vi "Mark Tool Error Result.vi"(8 "error in":errorcluster, 11 "response":string) -> (0 "error out":errorcluster, 3 "response out":string)   [LabVIEW 2020, in "MCP Server.lvlib"]
doc: "Marks the result of tools/call as a tool execution error when the tool VI itself reported an error.\n\nThe outputs of the tool are returned as one JSON object in the first text item of content. If one of the outputs is an error cluster (an object with status, code and source) whose status is true, the result gets \"isError\": true. The content is not changed.\n\nEvery other response is passed through."
uses:
  MCP Server.lvlib
  5611462b-074d-46fb-9f1a-e631b5fec0f0.vi
  <vilib>/JDP Science/JSONtext/Next JSON Value.vi
  <vilib>/JDP Science/JSONtext/String Subset.vi
  <vilib>/JDP Science/JSONtext/Parsing/Advance past next JSON Value (inlined COPY).vi
  <vilib>/JDP Science/JSONtext/Parsing/Advance past whitespace.vi
  <vilib>/JDP Science/JSONtext/Parsing/Advance past String.vi
  <vilib>/JDP Science/JSONtext/Parsing/Advance past Number.vi
  <vilib>/JDP Science/JSONtext/Parsing/Advance past Line Ending.vi
  <vilib>/JDP Science/JSONtext/Parsing/Parse Full Path or Item Name.vi
  <vilib>/JDP Science/JSONtext/Parsing/Advance past Array.vi
  <vilib>/JDP Science/JSONtext/Parsing/Advance past Object.vi
  <vilib>/JDP Science/JSONtext/support/Error Cluster From Code.vi
  <vilib>/JDP Science/JSONtext/Offset/Find Item Locations by Path.vi
  <vilib>/JDP Science/JSONtext/JSON text to Variant.vi
  <vilib>/JDP Science/JSONtext/LVClass Serializer/JSONtext LVClass Serializer.lvclass
  <vilib>/JDP Science/JSONtext/JSONtext.lvlib
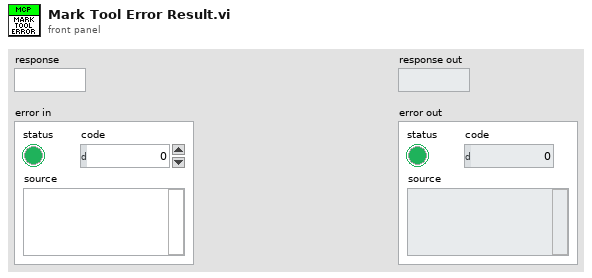
[diagram p1: front panel]
types:
  T1 = typedef "JSONtext.lvlib/JSON Value Type.ctl" = enum16{"Not a JSON Value", "JSON Object", "JSON Array", "String", "Number", "true", "false", "null"}
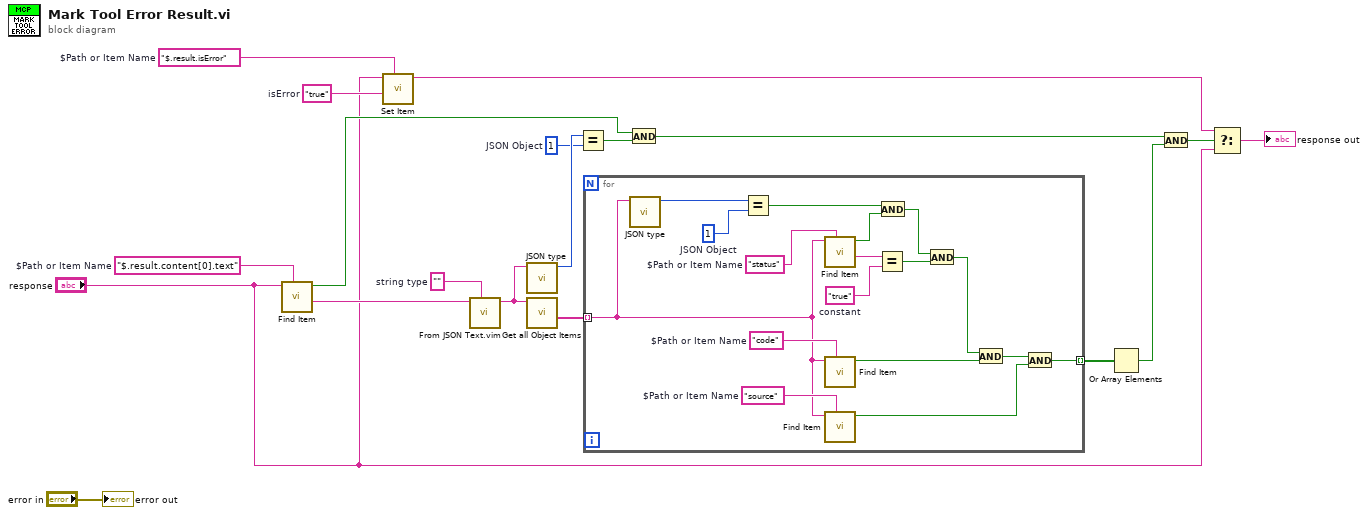
[diagram p0: block diagram]
diagram:
  w11 = "$.result.isError"  # $Path or Item Name
  w10 = "true"  # isError
  w15 = u16 1  # JSON Object
  w17 = ""  # string type
  w19 = "$.result.content[0].text"  # $Path or Item Name
  n1 = call <vilib>:"Find Item.vi"("$Path or Item Name"=w19, "JSON"="response") -> ("<JSON>"=w18:string, "Found"=w9:bool)  [unwired: 6 in, 2 out]
  n2 = call <vilib>:"Set Item.vi"("$Path or Item Name"=w11, "JSON to Insert"=w10, "JSON"="response") -> ("<JSON>"=w5:string)  [unwired: 5 in, 2 out]
  n3 = call "From JSON Text.vim"("Data Type and Default Value"=w17, "JSON"=w18) -> ("Data out"=w14:string)  [unwired: 8 in, 1 out]
  n4 = call <vilib>:"JSON type.vi"("JSON"=w14) -> ("JSON Value Type"=w16:T1)  [unwired: 9 in, 1 out]
  n5 = call <vilib>:"Get all Object Items.vi"("JSON"=w14) -> ("<JSON>"=w13:string[])  [unwired: 7 in, 3 out]
  n6 = Equal?(x=w16, y=w15) -> (x = y?=w8:bool)
  n7 = for {
    tunnel: w13 -> [w33] mode=indexing
    tunnel: [w20] -> w12 mode=indexing
    w29 = "true"  # constant
    w31 = u16 1  # JSON Object
    w34 = "source"  # $Path or Item Name
    w35 = "code"  # $Path or Item Name
    w36 = "status"  # $Path or Item Name
    n8 = call <vilib>:"JSON type.vi"("JSON"=w33) -> ("JSON Value Type"=w32:T1)  [unwired: 9 in, 1 out]
    n9 = Equal?(x=w32, y=w31) -> (x = y?=w28:bool)
    n10 = call <vilib>:"Find Item.vi"("$Path or Item Name"=w36, "JSON"=w33) -> ("<JSON>"=w30:string, "Found"=w27:bool)  [unwired: 6 in, 2 out]
    n11 = call <vilib>:"Find Item.vi"("$Path or Item Name"=w35, "JSON"=w33) -> ("Found"=w23:bool)  [unwired: 6 in, 3 out]
    n12 = call <vilib>:"Find Item.vi"("$Path or Item Name"=w34, "JSON"=w33) -> ("Found"=w21:bool)  [unwired: 6 in, 3 out]
    n13 = Equal?(x=w30, y=w29) -> (x = y?=w25:bool)
    n14 = And(x=w28, y=w27) -> (x .and. y?=w26:bool)
    n15 = And(x=w26, y=w25) -> (x .and. y?=w24:bool)
    n16 = And(x=w24, y=w23) -> (x .and. y?=w22:bool)
    n17 = And(x=w22, y=w21) -> (x .and. y?=w20:bool)
  }
  n18 = And(x=w9, y=w8) -> (x .and. y?=w7:bool)
  n19 = Or Array Elements(Boolean array=w12) -> (logical OR=w6:bool)
  n20 = And(x=w7, y=w6) -> (x .and. y?=w4:bool)
  n21 = Select(t=w5, s=w4, f="response") -> (s? t:f=→"response out":string)
  "error out" <- "error in"
